vi "exprparse.vi"(11 "Expression in":string) -> (1 "Placeholders":string[](array[string]), 2 "Tag Names":string[](array[string]), 3 "Expression out":string)   [LabVIEW 2020, in "Tag Expr.lvclass"]
doc: "Finds every ${TAG_NAME} in the expression and replaces it with a placeholder variable name that muParser accepts (TAG00, TAG01, ...). The same Tag used more than once gets the same placeholder.\n\nReturns the modified expression, the unique Tag names (in upper case) and their placeholders, in matching order.\n\nUsed by Construct."
uses:
  Tag Expr.lvclass
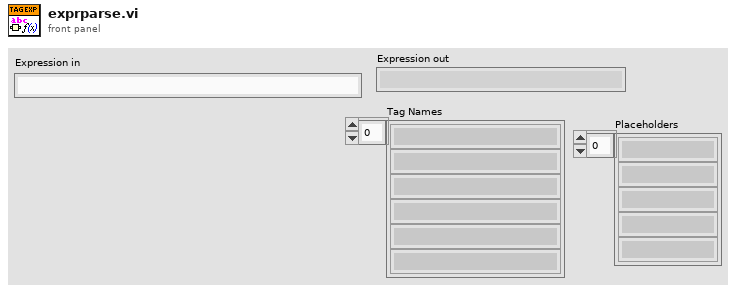
[diagram p1: front panel]
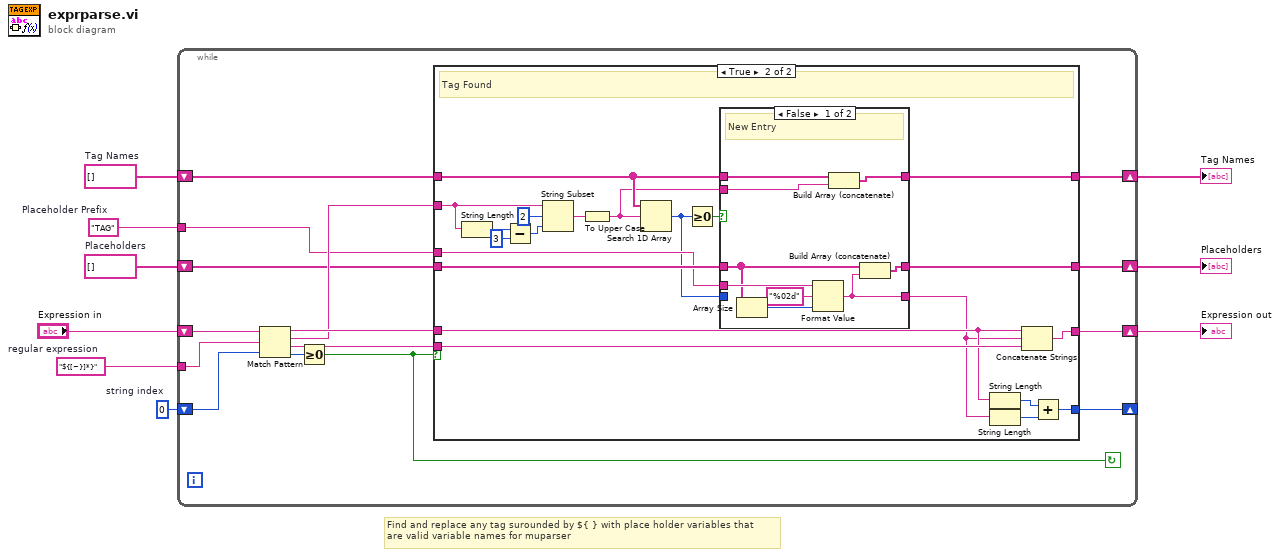
[diagram p0: block diagram]
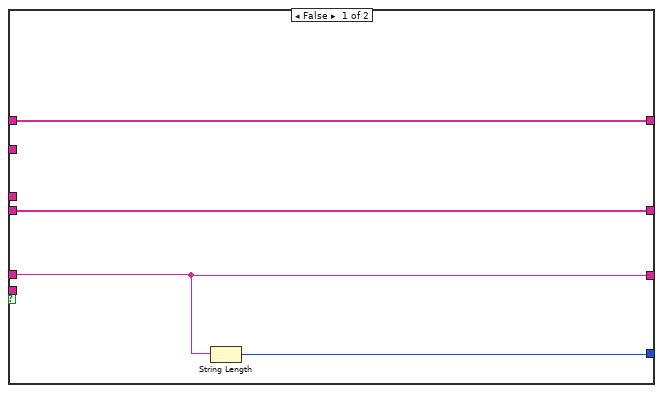
[diagram p2: hidden frame]
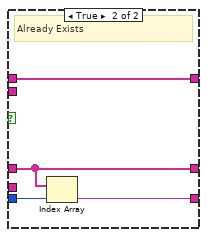
[diagram p3: hidden frame]
diagram:
  w3 = string[] []  # Placeholders
  w4 = string[] []  # Tag Names
  w8 = "${[~}]*}"  # regular expression
  w5 = "TAG"  # Placeholder Prefix
  w6 = 0  # string index
  # "Find and replace any tag surounded by ${ } with place holder variables that\nare valid variable names for muparser"
  n1 = while {
    shift-right: [w21] -> w7
    shift-left: "Expression in" -> [w24]
    tunnel: w8 -> [w23]
    shift-right: [w19] -> _
    shift-left: w6 -> [w18]
    tunnel: w5 -> [w12]
    shift-right: [w11] -> w2
    shift-left: w4 -> [w14]
    shift-right: [w10] -> w1
    shift-left: w3 -> [w13]
    stop <- w16 continue-if-true
    n2 = Match Pattern(string=w24, regular expression=w23, offset (0)=w18) -> (before substring=w20:string, match substring=w15:string, after substring=w22:string, offset past match=w17:i32)
    n3 = Greater Or Equal To 0?(x=w17) -> (x >= 0?=w16:bool)
    n4 = case shown="True" w16 {
      tunnel: w22 -> [_ w49]
      tunnel: [w27 w48] -> w21
      tunnel: w20 -> [w27 w47]
      tunnel: [w28 w44] -> w19
      tunnel: w15 -> [_ w39]
      tunnel: w14 -> [w26 w36]
      tunnel: w13 -> [w25 w33]
      tunnel: w12 -> [_ w32]
      tunnel: [w26 w34] -> w11
      tunnel: [w25 w31] -> w10
      frame False {
        n5 = String Length(string=w27) -> (length=w28:i32)
      }
      frame True {
        # "Tag Found"
        n6 = String Length(string=w39) -> (length=w41:i32)
        n7 = Subtract(x=w41, y=3) -> (x-y=w42:i32)
        n8 = String Subset(string=w39, offset (0)=2, length (rest)=w42) -> (substring=w38:string)
        n9 = To Upper Case(1:w38) -> (0:w35:string)
        n10 = Search 1D Array(1D array=w36, element=w35) -> (index of element=w29:i32)  [unwired: 1 in]
        n11 = Greater Or Equal To 0?(x=w29) -> (x >= 0?=w37:bool)
        n12 = case shown="False" w37 {
          tunnel: w36 -> [w58 w62]
          tunnel: w35 -> [w57 _]
          tunnel: [w56 w62] -> w34
          tunnel: w33 -> [w51 w61]
          tunnel: w32 -> [w55 _]
          tunnel: [w54 w61] -> w31
          tunnel: [w53 w59] -> w30
          tunnel: w29 -> [_ w60]
          frame False {
            # "New Entry"
            n13 = Array Size(array=w51) -> (size(s)=w50:i32)
            n14 = Format Value(string ("")=w55, format string="%02d", value (0)=w50) -> (output string=w53:string)
            n15 = Build Array (concatenate)(w58, w57) -> (w56:string[])
            n16 = Build Array (concatenate)(w51, w53) -> (w54:string[])
          }
          frame True {
            # "Already Exists"
            n17 = Index Array(array=w61, index=w60) -> (element=w59:string)
          }
        }
        n18 = String Length(string=w47) -> (length=w46:i32)
        n19 = String Length(string=w30) -> (length=w45:i32)
        n20 = Concatenate Strings(w47, w30, w49) -> (w48:string)
        n21 = Add(x=w46, y=w45) -> (x+y=w44:i32)
      }
    }
  }
  "Expression out" <- w7
  "Tag Names" <- w2
  "Placeholders" <- w1
